vi "Init.vi"(8 "error in (no error)":errorcluster, 11 "Data in":refnum<class "CTI_AnalogIn.lvclass">) -> (0 "error out":errorcluster, 3 "Data out":refnum<class "CTI_AnalogIn.lvclass">)   [LabVIEW 2021, in "CTI_AnalogIn.lvclass"]
doc: "Abstract Data Classes 2.1.1.13\nTim Streeter - TSA\nCopyright (c) 2025, TSA"
uses:
  CTI_AnalogIn.lvclass
  CTI_AnalogIn.lvclass/CTI_AnalogIn.ctl
  <vilib>/CTI/CTI Drivers/CTI/Session/Session.lvclass
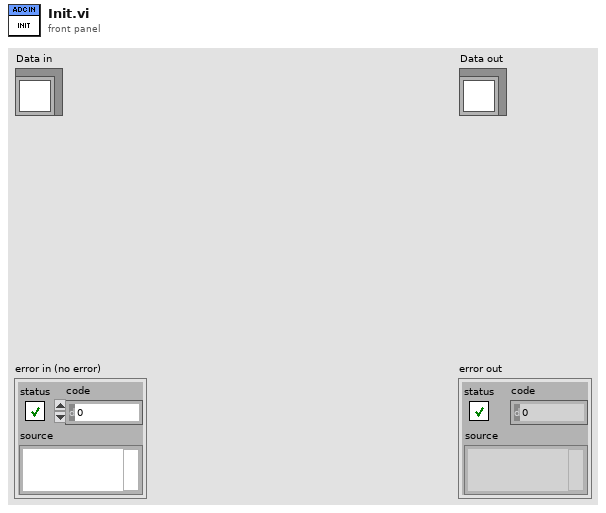
[diagram p1: front panel]
types:
  T1 = typedef "CTI.lvlib/ADC Number.ctl" = i8
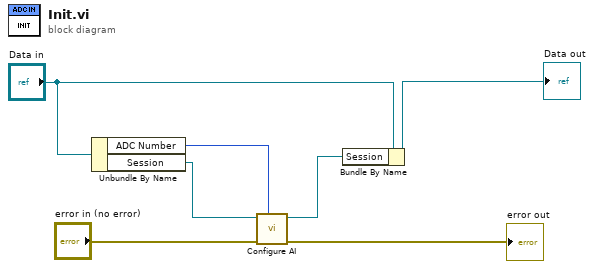
[diagram p0: block diagram]
diagram:
  n1 = Unbundle By Name("Data in") -> ("ADC Number"=w3:T1, "Session"=w4:refnum<class "Session.lvclass">)
  n2 = call <vilib>:"Configure AI.vi"("ADC #"=w3, "error in (no error)"="error in (no error)", "Session in"=w4) -> ("error out"=→"error out":errorcluster, "Session out"=w1:refnum<class "Session.lvclass">)  [unwired: 7 in]
  n3 = Bundle By Name(cluster="Data in", "Session"=w1) -> (→"Data out":refnum<class "CTI_AnalogIn.lvclass">)
